vi "Dynamic InputVoltage.vi"(8 "error in (no error)":errorcluster) -> (0 "error out":errorcluster)   [LabVIEW 2025]
uses:
  SubVIs/All test cluster.ctl
  SubVIs/All_enum_ctl.ctl
  SubVIs/Arduino_lamps.ctl
  <vilib>/numeric/Random Number (Range) U64.vi
  <vilib>/numeric/sub_Random U32.vi
  SubVIs/Lamps_global.vi
  <vilib>/Utility/file.llb/Write Delimited Spreadsheet (string).vi
  <instrlib>/BK Precision 9200 Series/BK Precision 9200 Series.lvlib
  <instrlib>/Keithley 2260B/Keithley 2260B.lvlib
panel:
  in  "ESP PORT":refnum<visa-resource-name>
  in  "No.Of Cycles":dbl=3.0
  out "Status":string
  in  "POWER SUPPLY":bool caption="Blank Button"
  out "Text name":string
  in  "COM PORT":refnum<visa-resource-name>
  in  "Start/Stop":bool caption="Slide Switch"
  in  "File Path:":path
  in  "FILENAME":string
  out "Table":string[][](table)
  out "Connected?":bool caption="Long Blank Button"
  out "Connected? 2":bool caption="Long Blank Button"
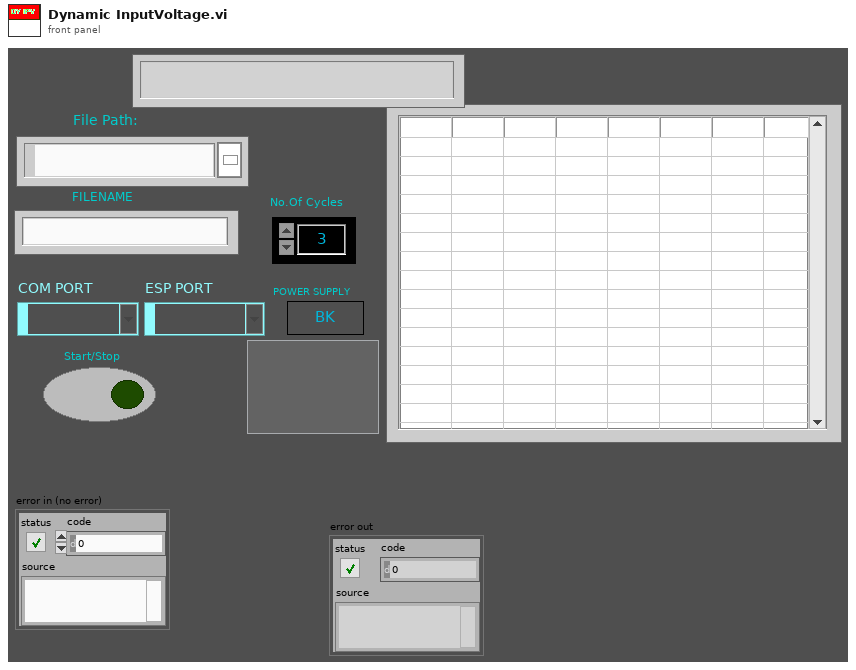
[diagram p1: front panel]
types:
  T1 = enum32{"Invalid", "Standard", "Closed", "Hidden", "Minimized", "Maximized"}
  T2 = typedef "All_enum_ctl.ctl" = enum16{"Init", "Poll", "Connect_esp32", "Connect", "check_start", "Start", "Set_Voltage", "On_relay", "Read_Voltage", "Off_Relay", "Next_Relay", "Next_Step", "Stop", "Store", "Error", "Exit"}
  T3 = typedef "All test cluster.ctl" = cluster{"FilePath":path, "Test Status":bool, "Start Volt":dbl, "End Volt":dbl, "Present Step":dbl, "Present Time(s)":dbl, "End Time":dbl, "Table":string[], "Intensity":string, "BK/Keith":bool, "COM":refnum<visa-resource-name>, "Next state":T2, "Step no.":dbl, "Start ms":u32, "ESP_COM":refnum<visa-resource-name>, "Relay_no":dbl, "Datas":string[]}
  T4 = typedef "Arduino_lamps.ctl" = enum16{"Init", "Poll", "Read", "Write", "Exit"}
  T5 = cluster{"Baud Rate":u32, "Parity":u16, "Data Bits":u16, "Stop Bits":u16, "Flow Control":u16}
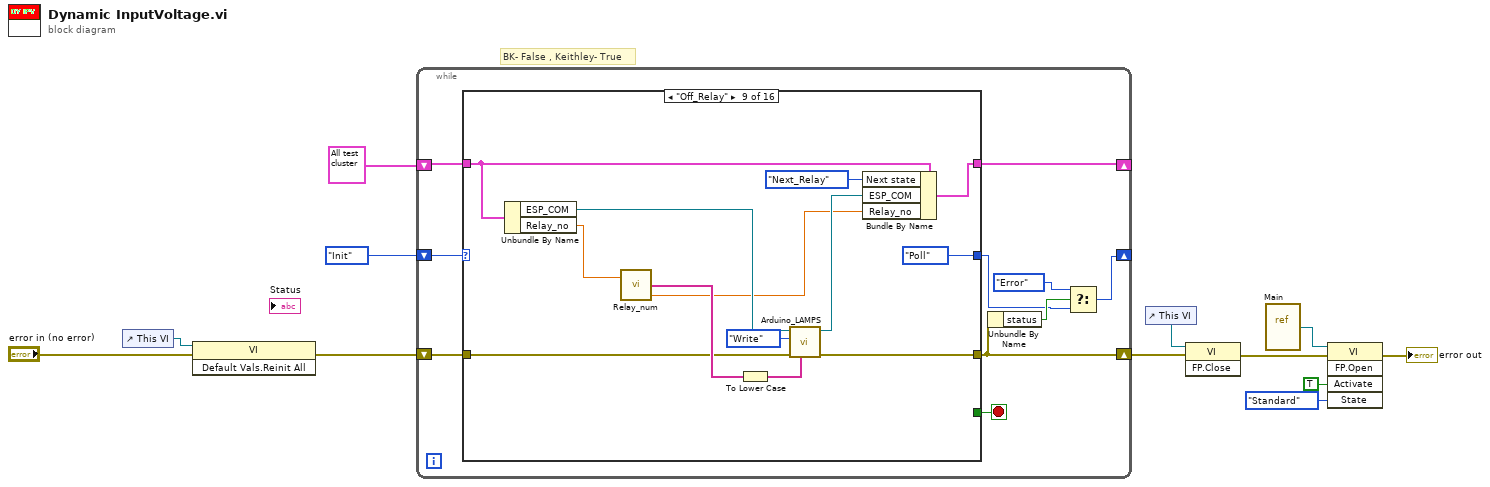
[diagram p0: block diagram]
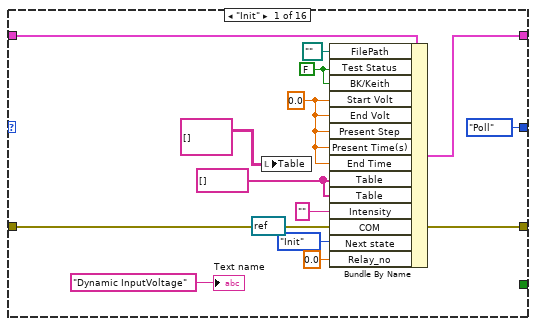
[diagram p2: hidden frame]
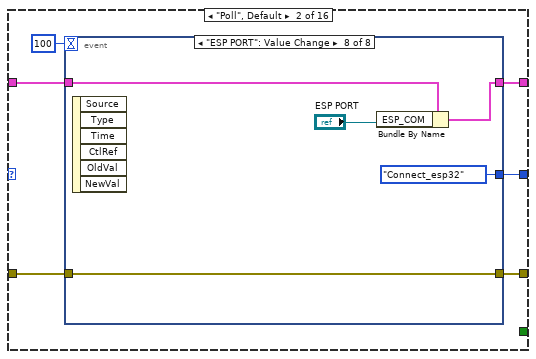
[diagram p3: hidden frame]
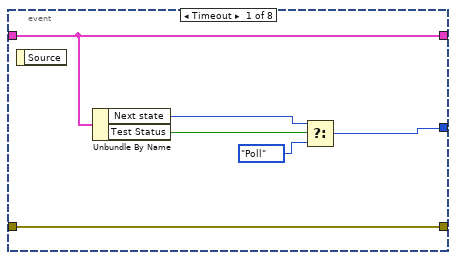
[diagram p4: hidden frame]
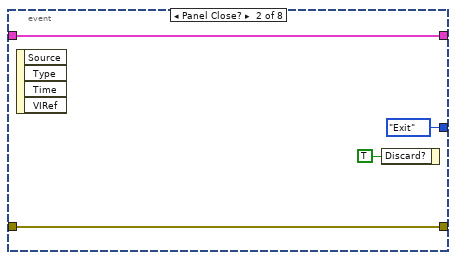
[diagram p5: hidden frame]
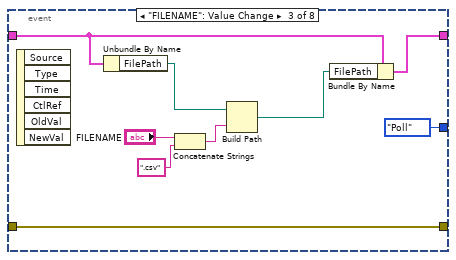
[diagram p6: hidden frame]
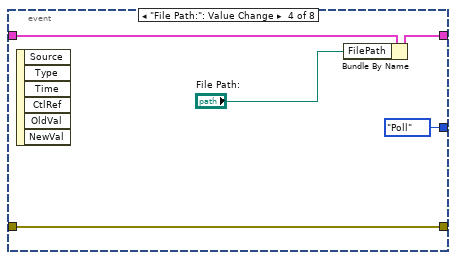
[diagram p7: hidden frame]
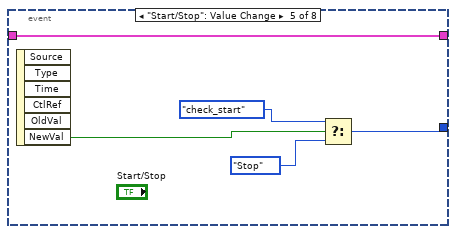
[diagram p8: hidden frame]
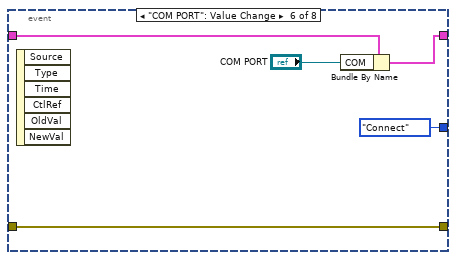
[diagram p9: hidden frame]
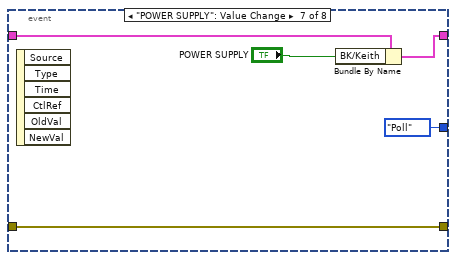
[diagram p10: hidden frame]
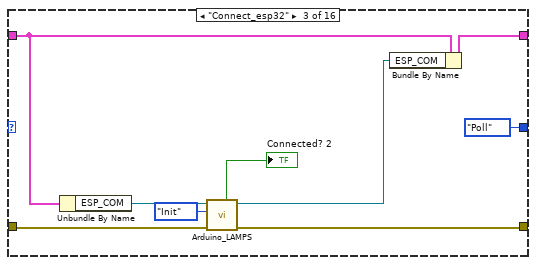
[diagram p11: hidden frame]
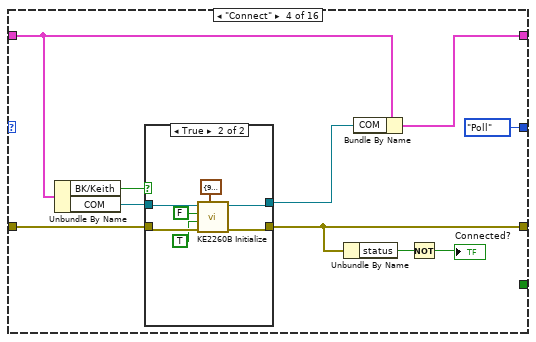
[diagram p12: hidden frame]
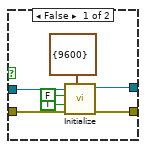
[diagram p13: hidden frame]
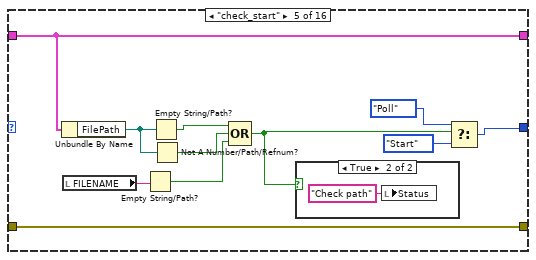
[diagram p14: hidden frame]
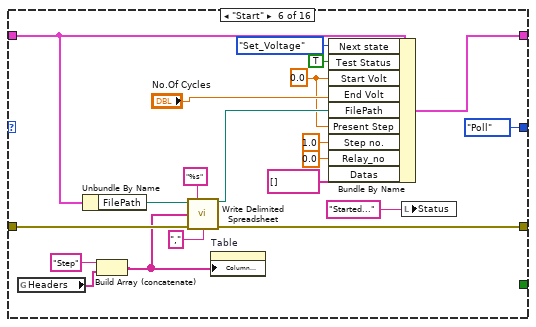
[diagram p16: hidden frame]
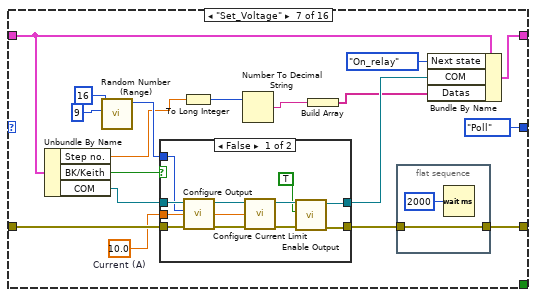
[diagram p17: hidden frame]
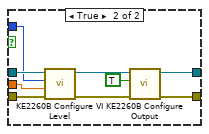
[diagram p18: hidden frame]
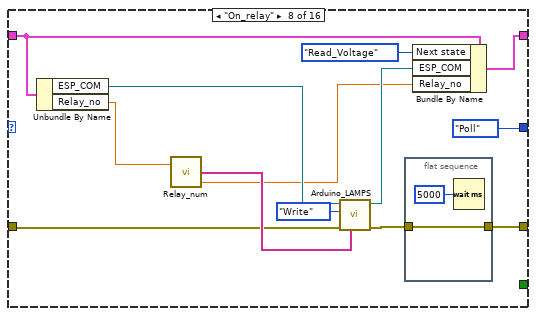
[diagram p19: hidden frame]
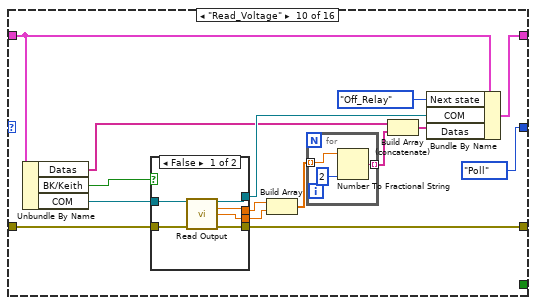
[diagram p20: hidden frame]
diagram:
  # "BK- False , Keithley- True"
  n1 = control-ref of="This VI"() -> (w12:refnum<vi>)
  n2 = invoke class="VI" method="Default Vals.Reinit All"(reference=w12, error in="error in (no error)") -> (error out=w10:errorcluster)  [unwired: 1 in, 2 out]
  n3 = while {
    shift-right: [w21] -> _
    shift-left: T3 {"FilePath"=path "", "Test Status"=FALSE, "Start Volt"=0.0, "End Volt"=0.0, "Present Step"=0.0, "Present Time(s)"=0.0, "End Time"=0.0, "Table"=[], "Intensity"="", "BK/Keith"=FALSE, "COM"="", "Next state"=enum."Init", "Step no."=0.0, "Start ms"=0, "ESP_COM"="", "Relay_no"=0.0, "Datas"=[]} -> [w20]
    shift-right: [w17] -> w2
    shift-left: w10 -> [w19]
    shift-right: [w13] -> _
    shift-left: All_enum_ctl."Init" -> [w22]
    stop <- w18 stop-if-true
    n4 = case shown="\"Off_Relay\"" w22 {
      tunnel: [w34 w39 w89 w97 w129 w150 w168 w195 w211 w229 w251 w282 w296 w310 w327 w345] -> w21
      tunnel: w20 -> [w36 w40 w91 w101 w129 w145 w167 w196 w212 w233 w252 w285 w292 w311 w330 w345]
      tunnel: w19 -> [w35 w42 w93 w105 w130 w147 w169 w193 w208 w234 w257 w286 w291 w315 w334 w348]
      tunnel: [w35 w41 w92 w100 w130 w146 w156 w192 w209 w232 w257 w279 w290 w315 w332 w346] -> w17
      tunnel: [All_enum_ctl."Poll" w37 All_enum_ctl."Poll" All_enum_ctl."Poll" w121 All_enum_ctl."Poll" All_enum_ctl."Poll" All_enum_ctl."Poll" All_enum_ctl."Poll" All_enum_ctl."Poll" All_enum_ctl."Poll" All_enum_ctl."Poll" All_enum_ctl."Poll" All_enum_ctl."Poll" All_enum_ctl."Poll" All_enum_ctl."Exit"] -> w14
      tunnel: [_ _ _ _ _ _ _ _ _ _ _ _ _ _ _ TRUE] -> w18
      frame "Init" {
        w25 = string[] [] ("Table")
        w32 = 0.0 ("Start Volt")
        w30 = FALSE ("Test Status")
        n5 = local write "Table"(string[][] [] ("Table")) -> ()
        n6 = Bundle By Name(cluster=w36, "FilePath"=path "", "Test Status"=w30, "BK/Keith"=w30, "Start Volt"=w32, "End Volt"=w32, "Present Step"=w32, "Present Time(s)"=w32, "End Time"=w32, "Table"=w25, "Table"=w25, "Intensity"="", "COM"=refnum<visa-resource-name> refnum, "Next state"=All_enum_ctl."Init" ("Last state"), "Relay_no"=0.0) -> (w34:T3)
        "Text name" <- "Dynamic InputVoltage"
      }
      frame "Poll", Default {
        n7 = event shown="[7] \"ESP PORT\": Value Change" {
          selector: _ -> [_ _ _ _ _ _ _ _]
          dyn-events: _ -> [_ _ _ _ _ _ _ _]
          timeout: 100 -> [_ _ _ _ _ _ _ _]
          tunnel: w42 -> [w48 w49 w61 w64 _ w72 w77 w86]
          tunnel: [w48 w49 w61 w64 _ w72 w77 w86] -> w41
          tunnel: w40 -> [w47 w50 w59 w66 w70 w76 w81 w85]
          tunnel: [w47 w50 w55 w63 w70 w75 w80 w84] -> w39
          tunnel: [w43 All_enum_ctl."Exit" ("f") All_enum_ctl."Poll" All_enum_ctl."Poll" w67 All_enum_ctl."Connect" ("f") All_enum_ctl."Poll" ("f") All_enum_ctl."Connect_esp32" ("f")] -> w37
          event Timeout {
            n8 = event-data() -> ()  [unwired: 1 in, 1 out]
            n9 = Unbundle By Name(w47) -> ("Next state"=w44:T2, "Test Status"=w46:bool)
            n10 = Select(t=w44, s=w46, f=All_enum_ctl."Poll") -> (s? t:f=w43:T2)
          }
          event Panel Close? {
            n11 = event-data() -> ()  [unwired: 1 in, 4 out]
            n12 = event-data("Discard?"=TRUE) -> ()  [unwired: 1 in, 1 out]
          }
          event "FILENAME": Value Change {
            n13 = event-data() -> ()  [unwired: 1 in, 6 out]
            n14 = Unbundle By Name(w59) -> ("FilePath"=w58:path)
            n15 = Concatenate Strings("FILENAME", ".csv" ("string")) -> (w57:string)
            n16 = Build Path(base path=w58, name or relative path=w57) -> (appended path=w54:path)
            n17 = Bundle By Name(cluster=w59, "FilePath"=w54) -> (w55:T3)
          }
          event "File Path:": Value Change {
            n18 = event-data() -> ()  [unwired: 1 in, 6 out]
            n19 = Bundle By Name(cluster=w66, "FilePath"="File Path:") -> (w63:T3)
          }
          event "Start/Stop": Value Change {
            n20 = event-data() -> ("NewVal"=w71:bool)  [unwired: 1 in, 5 out]
            n21 = Select(t=All_enum_ctl."check_start", s=w71, f=All_enum_ctl."Stop") -> (s? t:f=w67:T2)
          }
          event "COM PORT": Value Change {
            n22 = event-data() -> ()  [unwired: 1 in, 6 out]
            n23 = Bundle By Name(cluster=w76, "COM"="COM PORT") -> (w75:T3)
          }
          event "POWER SUPPLY": Value Change {
            n24 = event-data() -> ()  [unwired: 1 in, 6 out]
            n25 = Bundle By Name(cluster=w81, "BK/Keith"="POWER SUPPLY") -> (w80:T3)
          }
          event "ESP PORT": Value Change {
            n26 = event-data() -> ()  [unwired: 1 in, 6 out]
            n27 = Bundle By Name(cluster=w85, "ESP_COM"="ESP PORT") -> (w84:T3)
          }
        }
      }
      frame "Connect_esp32" {
        n28 = Unbundle By Name(w91) -> ("ESP_COM"=w94:refnum<visa-resource-name>)
        n29 = call "Arduino_LAMPS.vi"("error out"=w93, "Enum"=Arduino_lamps."Init", "VISA resource name"=w94) -> ("error out 2"=w92:errorcluster, "VISA out"=w88:refnum<visa-resource-name>, "status"=→"Connected? 2":bool)  [unwired: 4 in, 2 out]
        n30 = Bundle By Name(cluster=w91, "ESP_COM"=w88) -> (w89:T3)
      }
      frame "Connect" {
        n31 = Unbundle By Name(w101) -> ("BK/Keith"=w99:bool, "COM"=w98:refnum<visa-resource-name>)
        n32 = case shown="True" w99 {
          tunnel: w105 -> [w112 w119]
          tunnel: [w111 w118] -> w100
          tunnel: w98 -> [w110 w117]
          tunnel: [w106 w115] -> w96
          frame False {
            n33 = call <instrlib>:"Initialize.vi"("Serial Configuration"=cluster{"Baud Rate":u32} {"Baud Rate"=9600}, "error in (no error)"=w112, "Reset (True)"=TRUE, "ID Query (True)"=FALSE, "VISA resource name"=w110) -> ("error out"=w111:errorcluster, "VISA resource name out"=w106:refnum<visa-resource-name>)  [unwired: 5 in]
          }
          frame True {
            n34 = call <instrlib>:"KE2260B Initialize.vi"("Serial Configuration"=T5 {"Baud Rate"=9600, "Parity"=0, "Data Bits"=8, "Stop Bits"=10, "Flow Control"=0}, "error in (no error)"=w119, "Reset (True)"=TRUE, "ID Query (True)"=FALSE, "VISA resource name"=w117) -> ("error out"=w118:errorcluster, "VISA resource name out"=w115:refnum<visa-resource-name>)  [unwired: 5 in]
          }
        }
        n35 = Unbundle By Name(w100) -> ("status"=w104:bool)
        n36 = Bundle By Name(cluster=w101, "COM"=w96) -> (w97:T3)
        n37 = Not(x=w104) -> (.not. x?=→"Connected?":bool)
      }
      frame "check_start" {
        n38 = Unbundle By Name(w129) -> ("FilePath"=w127:path)
        n39 = local read "FILENAME"() -> (w128:string)
        n40 = Empty String/Path?(string/path=w128) -> (empty?=w124:bool)
        n41 = Empty String/Path?(string/path=w127) -> (empty?=w126:bool)
        n42 = Not A Number/Path/Refnum?(number/path/refnum=w127) -> (NaN/Path/Refnum?=w125:bool)
        n43 = Compound Arithmetic op=OR(w126, w125, w124) -> (w120:bool)
        n44 = case shown="True" w120 {
          frame False {
          }
          frame True {
            n45 = local write "Status"("Check path") -> ()
          }
        }
        n46 = Select(t=All_enum_ctl."Poll", s=w120, f=All_enum_ctl."Start") -> (s? t:f=w121:T2)
      }
      frame "Start" {
        w138 = 0.0 ("Start Volt")
        n47 = global read "Lamps_global.vi" "Headers"() -> (w135:string[])
        n48 = Unbundle By Name(w145) -> ("FilePath"=w144:path)
        n49 = Build Array (concatenate)("Step" ("String"), w135) -> (w132:string[])
        n50 = call-poly <vilib>:"Write Delimited Spreadsheet.vi"("file path (dialog if empty)"=w144, "format (%s)"="%s" ("format (%.3f)"), "1D data"=w132, "error in (no error)"=w147, "delimiter (\\t)"="," ("delimiter (\\t)")) -> ("new file path (Not A Path if cancelled)"=w141:path, "error out"=w146:errorcluster)  [unwired: 9 in]
        n51 = property on="Table" class="Tbl (strict)"("Column Headers[]"=w132) -> ()  [unwired: 2 in, 2 out]
        n52 = Bundle By Name(cluster=w145, "Next state"=All_enum_ctl."Set_Voltage" ("Last state"), "Test Status"=TRUE, "Start Volt"=w138, "End Volt"="No.Of Cycles", "FilePath"=w141, "Present Step"=w138, "Step no."=1.0, "Relay_no"=0.0, "Datas"=string[] []) -> (w150:T3)
        n53 = local write "Status"("Started...") -> ()
      }
      frame "Set_Voltage" {
        w162 = 10.0  # Current (A)
        n54 = Unbundle By Name(w167) -> ("Step no."=w153:dbl, "BK/Keith"=w163:bool, "COM"=w166:refnum<visa-resource-name>)
        n55 = call-poly <vilib>:"Random Number (Range).vi"("lower bound (0)"=u64 9, "upper bound (100)"=u64 16) -> ("number"=w158:u64)  [unwired: 9 in]
        n56 = case shown="False" w163 {
          tunnel: w169 -> [w175 w191]
          tunnel: [w182 w190] -> w157
          tunnel: w166 -> [w180 w188]
          tunnel: [w181 w186] -> w165
          tunnel: w158 -> [w179 w184]
          tunnel: w162 -> [w173 w183]
          frame False {
            n57 = call <instrlib>:"Configure Output.vi"("error in (no error)"=w175, "Voltage Level (0.0 V)"=w179, "VISA resource name"=w180) -> ("error out"=w176:errorcluster, "VISA resource name out"=w174:refnum<visa-resource-name>)  [unwired: 7 in]
            n58 = call <instrlib>:"Configure Current Limit.vi"("error in (no error)"=w176, "Current Limit (0.0 A)"=w173, "VISA resource name"=w174) -> ("error out"=w178:errorcluster, "VISA resource name out"=w177:refnum<visa-resource-name>)  [unwired: 7 in]
            n59 = call <instrlib>:"Enable Output.vi"("error in (no error)"=w178, "Enable Output (F: False)"=TRUE, "VISA resource name"=w177) -> ("error out"=w182:errorcluster, "VISA resource name out"=w181:refnum<visa-resource-name>)  [unwired: 7 in]
          }
          frame True {
            n60 = call <instrlib>:"KE2260B Configure VI Level.vi"("error in (no error)"=w191, "Current Level (0.000 A)"=w183, "Voltage Level (0.000 V)"=w184, "VISA resource name"=w188) -> ("error out"=w189:errorcluster, "VISA resource name out"=w187:refnum<visa-resource-name>)  [unwired: 6 in]
            n61 = call <instrlib>:"KE2260B Configure Output.vi"("error in (no error)"=w189, "Enable Output (T: Enable)"=TRUE, "VISA resource name"=w187) -> ("error out"=w190:errorcluster, "VISA resource name out"=w186:refnum<visa-resource-name>)  [unwired: 7 in]
          }
        }
        n62 = To Long Integer(number=w153) -> (32bit integer=w155:i32)
        n63 = Number To Decimal String(number=w155) -> (decimal integer string=w154:string)  [unwired: 1 in]
        n64 = Build Array(w154) -> (w152:string[])
        n65 = flat-sequence {
          tunnel: w157 -> [w170]
          tunnel: [w170] -> w156
          frame #0 {
            n66 = Wait (ms)(milliseconds to wait=u32 2000) -> ()  [unwired: 1 out]
          }
        }
        n67 = Bundle By Name(cluster=w167, "Next state"=All_enum_ctl."On_relay", "COM"=w165, "Datas"=w152) -> (w168:T3)
      }
      frame "On_relay" {
        n68 = Unbundle By Name(w196) -> ("ESP_COM"=w204:refnum<visa-resource-name>, "Relay_no"=w199:dbl)
        n69 = call "Relay_num.vi"("Relay_no."=w199) -> ("Relay"=w198:string[], "Relay_no.out"=w197:dbl)  [unwired: 1 in, 1 out]
        n70 = call "Arduino_LAMPS.vi"("DO's"=w198, "error out"=w193, "Enum"=Arduino_lamps."Write", "VISA resource name"=w204) -> ("error out 2"=w200:errorcluster, "VISA out"=w202:refnum<visa-resource-name>)  [unwired: 3 in, 3 out]
        n71 = flat-sequence {
          tunnel: w200 -> [w206]
          tunnel: [w206] -> w192
          frame #0 {
            n72 = Wait (ms)(milliseconds to wait=u32 5000) -> ()  [unwired: 1 out]
          }
        }
        n73 = Bundle By Name(cluster=w196, "Next state"=All_enum_ctl."Read_Voltage", "ESP_COM"=w202, "Relay_no"=w197) -> (w195:T3)
      }
      frame "Off_Relay" {
        n74 = Unbundle By Name(w212) -> ("ESP_COM"=w219:refnum<visa-resource-name>, "Relay_no"=w215:dbl)
        n75 = call "Relay_num.vi"("Relay_no."=w215) -> ("Relay"=w214:string[], "Relay_no.out"=w213:dbl)  [unwired: 1 in, 1 out]
        n76 = To Lower Case(string=w214) -> (all lower case string=w207:string[])
        n77 = call "Arduino_LAMPS.vi"("DO's"=w207, "error out"=w208, "Enum"=Arduino_lamps."Write", "VISA resource name"=w219) -> ("error out 2"=w209:errorcluster, "VISA out"=w217:refnum<visa-resource-name>)  [unwired: 3 in, 3 out]
        n78 = Bundle By Name(cluster=w212, "Next state"=All_enum_ctl."Next_Relay", "ESP_COM"=w217, "Relay_no"=w213) -> (w211:T3)
      }
      frame "Read_Voltage" {
        n79 = Unbundle By Name(w233) -> ("Datas"=w220:string[], "BK/Keith"=w230:bool, "COM"=w231:refnum<visa-resource-name>)
        n80 = case shown="False" w230 {
          tunnel: w234 -> [w243 w249]
          tunnel: [w242 w248] -> w232
          tunnel: w231 -> [w241 w246]
          tunnel: [w240 w247] -> w228
          tunnel: [w239 w245] -> w225
          tunnel: [w238 w244] -> w224
          frame False {
            n81 = call <instrlib>:"Read Output.vi"("VISA resource name"=w241, "error in (no error)"=w243) -> ("VISA resource name out"=w240:refnum<visa-resource-name>, "Actual Voltage Level (V)"=w239:dbl, "Actual Current Level (A)"=w238:dbl, "error out"=w242:errorcluster)  [unwired: 9 in, 1 out]
          }
          frame True {
            n82 = call <instrlib>:"KE2260B Read Output.vi"("error in (no error)"=w249, "VISA resource name"=w246) -> ("error out"=w248:errorcluster, "Actual Current Level (A)"=w244:dbl, "Actual Voltage Level (V)"=w245:dbl, "VISA resource name out"=w247:refnum<visa-resource-name>)  [unwired: 6 in]
          }
        }
        n83 = Build Array(w225, w224) -> (w223:dbl[])
        n84 = for {
          tunnel: w223 -> [w236] mode=indexing
          tunnel: [w235] -> w222 mode=indexing
          n85 = Number To Fractional String(number=w236, precision (6)=i16 2) -> (F-format string=w235:string)  [unwired: 2 in]
        }
        n86 = Build Array (concatenate)(w220, w222) -> (w221:string[])
        n87 = Bundle By Name(cluster=w233, "Next state"=All_enum_ctl."Off_Relay", "COM"=w228, "Datas"=w221) -> (w229:T3)
      }
      frame "Next_Relay" {
        n88 = Unbundle By Name(w252) -> ("Relay_no"=w256:dbl, "Datas"=w253:string[])
        n89 = call "Relay_num.vi"("Relay_no."=w256) -> ("x = y?"=w255:bool, "Relay_no.out"=w254:dbl)  [unwired: 1 in, 1 out]
        n90 = case shown="True" w255 {
          tunnel: [w267 w272] -> w251
          tunnel: w252 -> [w266 w271]
          tunnel: w254 -> [w264 _]
          tunnel: w253 -> [w258 w268]
          frame False {
            n91 = local read "Table"() -> (w262:string[][])
            n92 = Increment(x=w264) -> (x+1=w263:dbl)
            n93 = Array Size(array=w262) -> (size(s)=w260:i32[])
            n94 = Index Array(array=w260) -> (element=w259:i32)  [unwired: 1 in]
            n95 = Bundle By Name(cluster=w266, "Next state"=All_enum_ctl."On_relay", "Relay_no"=w263, "Datas"=w258) -> (w267:T3)
            n96 = Replace Array Subset(array=w262, new element=w258, index (row)=w259) -> (w261:string[][])  [unwired: 1 in]
            n97 = local write "Table"(w261) -> ()
          }
          frame True {
            n98 = Bundle By Name(cluster=w271, "Next state"=All_enum_ctl."Store", "Relay_no"=0.0, "Table"=w268) -> (w272:T3)
          }
        }
      }
      frame "Store" {
        n99 = Unbundle By Name(w285) -> ("Table"=w276:string[], "FilePath"=w278:path)
        n100 = local read "Table"() -> (w284:string[][])
        n101 = Build Array (concatenate)(w284, w276) -> (→"Table":string[][])
        n102 = call-poly <vilib>:"Write Delimited Spreadsheet.vi"("file path (dialog if empty)"=w278, "format (%s)"="%s", "1D data"=w276, "append to file? (new file:F)"=TRUE, "error in (no error)"=w286, "delimiter (\\t)"="," ("delimiter (\\t)")) -> ("new file path (Not A Path if cancelled)"=w275:path, "error out"=w279:errorcluster)  [unwired: 8 in]
        n103 = Bundle By Name(cluster=w285, "Next state"=All_enum_ctl."Next_Step", "FilePath"=w275) -> (w282:T3)
      }
      frame "Stop" {
        n104 = Unbundle By Name(w292) -> ("BK/Keith"=w293:bool, "COM"=w294:refnum<visa-resource-name>)
        n105 = case shown="False" w293 {
          tunnel: w291 -> [w300 w306]
          tunnel: [w302 w307] -> w290
          tunnel: w294 -> [w299 w305]
          tunnel: [w301 w304] -> w289
          frame False {
            n106 = call <instrlib>:"Enable Output.vi"("error in (no error)"=w300, "Enable Output (F: False)"=FALSE, "VISA resource name"=w299) -> ("error out"=w302:errorcluster, "VISA resource name out"=w301:refnum<visa-resource-name>)  [unwired: 7 in]
          }
          frame True {
            n107 = call <instrlib>:"KE2260B Configure Output.vi"("error in (no error)"=w306, "Enable Output (T: Enable)"=FALSE, "VISA resource name"=w305) -> ("error out"=w307:errorcluster, "VISA resource name out"=w304:refnum<visa-resource-name>)  [unwired: 7 in]
          }
        }
        n108 = local write "Start/Stop"(FALSE ("Start/Stop")) -> ()
        n109 = Bundle By Name(cluster=w292, "Test Status"=FALSE, "COM"=w289) -> (w296:T3)
        n110 = local write "Status"("Test Stopped....") -> ()
      }
      frame "Next_Step" {
        n111 = Unbundle By Name(w311) -> ("Present Step"=w312:dbl, "End Volt"=w313:dbl, "Step no."=w308:dbl)
        n112 = Greater Or Equal?(x=w312, y=w313) -> (x >= y?=w314:bool)
        n113 = case shown="False" w314 {
          tunnel: w312 -> [w317 _]
          tunnel: w311 -> [w322 w325]
          tunnel: [w321 w324] -> w310
          tunnel: w308 -> [w319 _]
          frame False {
            n114 = Increment(x=w319) -> (x+1=w318:dbl)
            n115 = Increment(x=w317) -> (x+1=w316:dbl)
            n116 = Bundle By Name(cluster=w322, "Next state"=All_enum_ctl."Set_Voltage", "Present Step"=w316, "Step no."=w318) -> (w321:T3)
          }
          frame True {
            n117 = Bundle By Name(cluster=w325, "Next state"=All_enum_ctl."Stop") -> (w324:T3)
          }
        }
      }
      frame "Error" {
        n118 = Unbundle By Name(w330) -> ("BK/Keith"=w328:bool, "COM"=w329:refnum<visa-resource-name>)
        n119 = case shown="False" w328 {
          tunnel: w334 -> [w337 w342]
          tunnel: [w338 w341] -> w331
          tunnel: w329 -> [w336 w340]
          tunnel: [w335 w339] -> w326
          frame False {
            n120 = call <instrlib>:"Reset.vi"("error in (no error)"=w337, "VISA resource name"=w336) -> ("error out"=w338:errorcluster, "VISA resource name out"=w335:refnum<visa-resource-name>)  [unwired: 8 in]
          }
          frame True {
            n121 = call <instrlib>:"KE2260B Reset.vi"("error in (no error)"=w342, "VISA resource name"=w340) -> ("error out"=w341:errorcluster, "VISA resource name out"=w339:refnum<visa-resource-name>)  [unwired: 8 in]
          }
        }
        n122 = call <vilib>:"Clear Errors.vi"("error in (no error)"=w331) -> ("error out"=w332:errorcluster)  [unwired: 5 in, 1 out]
        n123 = Bundle By Name(cluster=w330, "COM"=w326) -> (w327:T3)
      }
      frame "Exit" {
        n124 = Unbundle By Name(w345) -> ("ESP_COM"=w343:refnum<visa-resource-name>, "BK/Keith"=w349:bool, "COM"=w350:refnum<visa-resource-name>)
        n125 = case shown="False" w349 {
          tunnel: w348 -> [w355 w358]
          tunnel: [w354 w357] -> w347
          tunnel: w350 -> [w353 w356]
          frame False {
            n126 = call <instrlib>:"Close.vi"("error in (no error)"=w355, "VISA resource name"=w353) -> ("error out"=w354:errorcluster)  [unwired: 9 in]
          }
          frame True {
            n127 = call <instrlib>:"KE2260B Close.vi"("error in (no error)"=w358, "VISA resource name"=w356) -> ("error out"=w357:errorcluster)  [unwired: 9 in]
          }
        }
        n128 = VISA Close(VISA resource name=w343, error in (no error)=w347) -> (error out=w344:errorcluster)
        n129 = call <vilib>:"Clear Errors.vi"("error in (no error)"=w344) -> ("error out"=w346:errorcluster)  [unwired: 5 in, 1 out]
      }
    }
    n130 = Unbundle By Name(w17) -> ("status"=w16:bool)
    n131 = Select(t=All_enum_ctl."Error", s=w16, f=w14) -> (s? t:f=w13:T2)
  }
  n132 = control-ref of="This VI"() -> (w3:refnum<vi>)
  n133 = invoke class="VI" method="FP.Close"(reference=w3, error in=w2) -> (error out=w1:errorcluster)  [unwired: 1 in, 2 out]
  n134 = vi-ref "Main.vi"() -> (w7:refnum<vi>)
  n135 = invoke class="VI" method="FP.Open"(reference=w7, error in=w1, "Activate"=TRUE ("Activate?"), "State"=T1."Standard") -> (error out=→"error out":errorcluster)  [unwired: 1 in, 4 out]
